vi "NanonisGetScanOffset.vi"(8 "error in (no error)":errorcluster, 11 "String input":string="string test") -> (0 "error out":errorcluster, 3 "String output":string)   [LabVIEW 2011]
uses:
  <userlib>/Nanonis Prog Interface/Nanonis Prog Interface.lvlib
panel:
  out "Application ref out":refnum<vi>
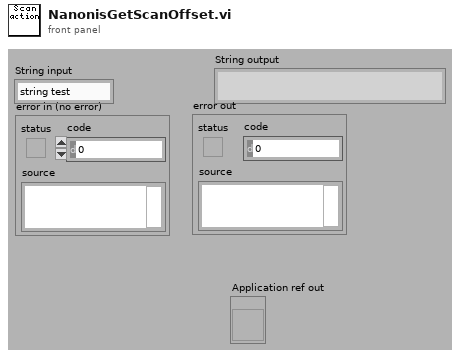
[diagram p1: front panel]
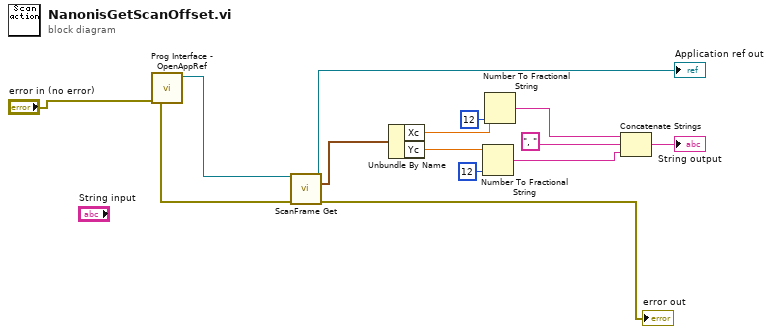
[diagram p0: block diagram]
diagram:
  n1 = call <userlib>:"Prog Interface - OpenAppRef.vi"("Error in (no error)"="error in (no error)") -> ("Error out"=w13:errorcluster, "Application reference"=w12:refnum<vi>)  [unwired: 5 in]
  n2 = call "ScanFrame Get.vi"("Application ref in"=w12, "error in (no error)"=w13) -> ("Application ref out"=→"Application ref out":refnum<vi>, "Center coordinates (m)"=w10:cluster{"Xc":sgl, "Yc":sgl}, "error out"=→"error out":errorcluster)  [unwired: 9 in, 2 out]
  n3 = Unbundle By Name(w10) -> ("Xc"=w9:sgl, "Yc"=w6:sgl)
  n4 = Number To Fractional String(number=w6, precision (6)=12) -> (F-format string=w3:string)  [unwired: 2 in]
  n5 = Number To Fractional String(number=w9, precision (6)=12) -> (F-format string=w5:string)  [unwired: 2 in]
  n6 = Concatenate Strings(w5, ", ", w3) -> (→"String output":string)
